vi "create.vi"(6 "Assets":string[](array[string]), 8 "error in (no error)":errorcluster, 9 "Start Time":timestamp format="%<%x %.3X>T", 10 "Title":string, 11 "Nominal Client":refnum<class "Nominal Client.lvclass">) -> (0 "error out":errorcluster, 3 "Run out":refnum<class "Run.lvclass">)   [LabVIEW 2020, in "Run.lvclass"]
uses:
  Run.lvclass
  Nominal Client/Nominal Client.lvclass
  Nominal Client/Nominal Client.lvclass/Nominal Client.ctl
  nominal types/workspace/workspace.lvclass/workspace.ctl
  Nominal Client/workspace.get.vi
  <vilib>/JDP Science/JSONtext/Merge into Object.vi
  Nominal Client/workspace.add_to_payload.vi/88650e10-de3e-481c-85db-71cb0fdf4485.vi
  nominal types/workspace/rid.get.vi
  Nominal Client/trace.payload_received.vi
  Nominal Client/error.vi
  Nominal Client/trace.payload_sent.vi
  Nominal Client/create.authorization_header.vi
  Nominal Client/trace.calling_method.vi
  Nominal Client/error.vi/859f8e04-e495-489b-b5b4-7ac163f56130.vi
  <vilib>/JDP Science/JDP Science Common Utilities/Trim Whitespace__JDP.vi
  <vilib>/AdvancedString/1D String Array to Delimited String.vi
  Nominal Client/api_token.get.vi
  <vilib>/JDP Science/JSONtext/Variant to JSON Text.vi
  <vilib>/JDP Science/JSONtext/Get all Object Items.vi
  <vilib>/JDP Science/JSONtext/Set Multiple Object Items.vi
  <vilib>/Utility/libraryn.llb/Get File Extension.vi
  Nominal Client/log_file.write.vi
  submodules/reqwest-labview/lv-src/reqwest/post.vi
  <vilib>/Utility/error.llb/Error Cluster From Error Code.vi
  <vilib>/JDP Science/JSONtext/JSON text to Variant.vi
  <vilib>/JDP Science/JSONtext/LVClass Serializer/JSONtext LVClass Serializer.lvclass
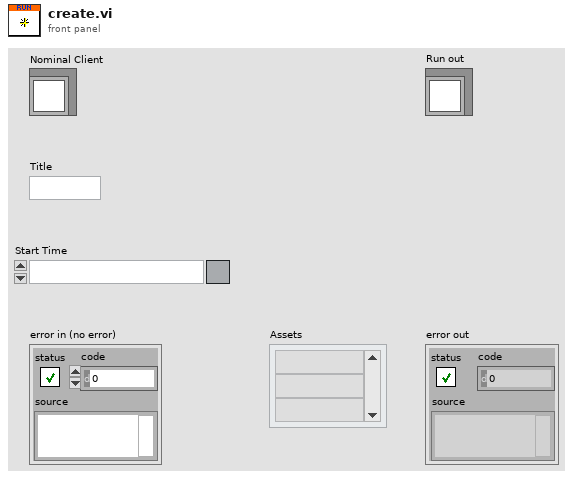
[diagram p1: front panel]
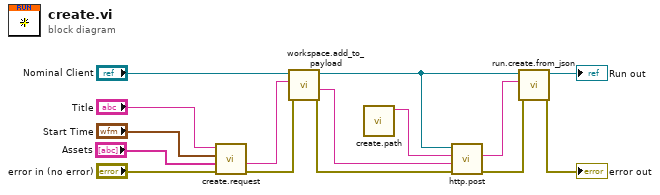
[diagram p0: block diagram]
diagram:
  n1 = call "create.request.vi"("error in"="error in (no error)", "Assets"="Assets", "Start Time"="Start Time", "Title"="Title") -> ("error out"=w3:errorcluster, "Request"=w4:string)  [unwired: 6 in]
  n2 = call "workspace.add_to_payload.vi"("error in"=w3, "JSON payload in"=w4, "Nominal Client in"="Nominal Client") -> ("error out"=w2:errorcluster, "JSON payload out"=w1:string, "Nominal Client out"=w5:refnum<class "Nominal Client.lvclass">)  [unwired: 6 in]
  n3 = call "create.path.vi"() -> ("Path"=w12:string)  [unwired: 11 in]
  n4 = call "http.post.vi"("error in"=w2, "Request body"=w1, "Path"=w12, "Nominal Client in"=w5) -> ("error out"=w9:errorcluster, "Response"=w10:string)  [unwired: 5 in, 1 out]
  n5 = call "run.create.from_json.vi"("error in"=w9, "JSON"=w10, "Nominal Client"=w5) -> ("error out"=→"error out":errorcluster, "Run out"=→"Run out":refnum<class "Run.lvclass">)  [unwired: 7 in]
